vi "TCP Server Connection Process Core.vi"(10 "TCP Server Refnum":refnum<class "JKI TCP Server.lvclass">, 11 "Self VI Refnum":refnum<vi>) -> ()   [LabVIEW 2020, in "JKI TCP Server.lvclass"]
uses:
  JKI TCP Server.lvclass
  JKI TCP Server.lvclass/JKI TCP Server.ctl
panel:
  # "This VI Must Be Reentrant if multiple *connections* are to be created."
  # "Copyright © 2004-2022 JKI. All rights reserved.\n\nAuthor: JKI [info@jki.net]\n\nThis library is provided \"AS IS\" ,WITHOUT WARRANTIES OR \nCONDITIONS OF ANY KIND, either express or implied.\n\nJKI -- http://www.jki.net"
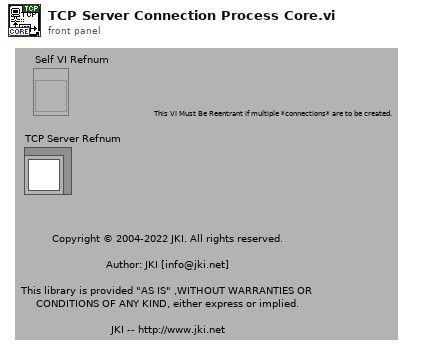
[diagram p1: front panel]
types:
  T1 = typedef "JKI TCP Server.lvclass/TCP Server Connection Info Cluster.ctl" = cluster{"connection ID":refnum<k5>, "Remote Address":string, "remote port":u16, "connection start time":u32}
  T2 = typedef "JKI TCP Server.lvclass/TCP Server Handler RefNum.ctl" = refnum<vi>
  T3 = cluster{"Connection Process VI Refnum":refnum<vi>, "TCP Handler VI RefNum":T2}
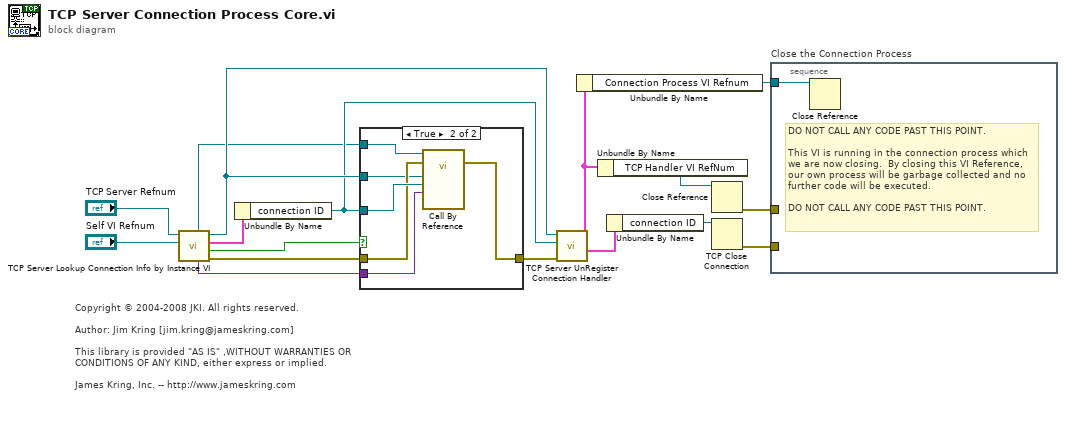
[diagram p0: block diagram]
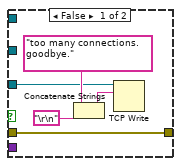
[diagram p2: hidden frame]
diagram:
  # "Copyright © 2004-2008 JKI. All rights reserved.\n\nAuthor: Jim Kring [jim.kring@jameskring.com]\n\nThis library is provided \"AS IS\" ,WITHOUT WARRANTIES OR \nCONDITIONS OF ANY KIND, either express or implied.\n\nJames Kring, Inc. -- http://www.jameskring.com"
  n1 = call "TCP Server Lookup Connection Info by Instance VI.vi"("Instance VI Refnum"="Self VI Refnum", "TCP Server"="TCP Server Refnum") -> ("error out"=w15:errorcluster, "OK to Start New Handler?"=w16:bool, "Connection Info"=w11:T1, "TCP Server out"=w17:refnum<class "JKI TCP Server.lvclass">, "Additional Data"=w1:variant, "Handler VI RefNum"=w12:T2)  [unwired: 4 in]
  n2 = Unbundle By Name(w11) -> ("connection ID"=w14:refnum<k5>)
  n3 = case shown="True" w16 {
    tunnel: w12 -> [_ w28]
    tunnel: [w22 w25] -> w13
    tunnel: w14 -> [w18 w27]
    tunnel: w15 -> [w22 w26]
    tunnel: w17 -> [_ w24]
    tunnel: w1 -> [_ w23]
    frame False {
      n4 = Concatenate Strings("too many connections.  goodbye." ("data in"), "\r\n") -> (w21:string)
      n5 = TCP Write(connection ID=w18, data in=w21) -> ()  [unwired: 2 in, 3 out]
    }
    frame True {
      n6 = call-by-ref "?"(reference=w28, error in=w26, "Additional Data"=w23, "connection ID"=w27, "TCP Server Refnum"=w24) -> (error out=w25:errorcluster)  [unwired: 9 in, 1 out]
    }
  }
  n7 = call "TCP Server UnRegister Connection Handler.vi"("error in (no error)"=w13, "connection ID"=w14, "TCP Server RefNum"=w17) -> ("Connection Info"=w8:T1, "VI References"=w3:T3)  [unwired: 6 in, 1 out]
  n8 = Unbundle By Name(w3) -> ("Connection Process VI Refnum"=w4:refnum<vi>)
  n9 = Unbundle By Name(w3) -> ("TCP Handler VI RefNum"=w2:T2)
  n10 = Unbundle By Name(w8) -> ("connection ID"=w7:refnum<k5>)
  n11 = Close Reference(reference=w2) -> (error out=w5:errorcluster)  [unwired: 1 in]
  n12 = TCP Close Connection(connection ID=w7) -> (error out=w6:errorcluster)  [unwired: 2 in, 1 out]
  n13 = stacked-sequence "Close the Connection Process" {
    tunnel: w4 -> [w29]
    tunnel: w6 -> [_]
    tunnel: w5 -> [_]
    frame #0 {
      # "DO NOT CALL ANY CODE PAST THIS POINT.\n\nThis VI is running in the connection process which we are now closing.  By closing this VI Reference, our own process will be garbage collected and no further code will be executed.\n\nDO NOT CALL ANY CODE PAST THIS POINT."
      n14 = Close Reference(reference=w29) -> ()  [unwired: 1 in, 1 out]
    }
  }
